vi "_Raise Nav Complete Event.vi"(4 "WebView2.lvlib:WebView2 Control.lvclass":refnum<class "WebView2 Control.lvclass">, 5 "Event Data":cluster{"sender":refnum<k24>, "e":refnum<k24>}, 6 "Control Ref":refnum<k24>, 7 "Event Common Data":T1) -> ()   [LabVIEW 2020, in "WebView2.lvlib" / "WebView2 Control.lvclass"]
uses:
  WebView2 Control.lvclass
  E:/Labview/LV 2023/PPL/PPL Builder/Libs/LV-WebView2/Source/Libs/Microsoft.Web.WebView2.Core.dll
  Libs/Microsoft.Web.WebView2.Core.dll
  WebView2 Control.lvclass/WebView2 Control.ctl
  WebView2 Event Filter Interface/WebView2 Event Filter Interface.lvclass
  Navigation Event Data.ctl
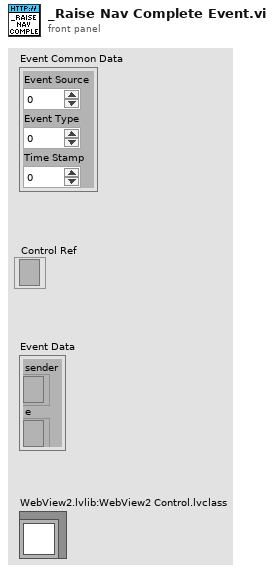
[diagram p1: front panel]
types:
  T1 = cluster{"Event Source":i32, "Event Type":u32, "Time Stamp":u32}
  T2 = typedef "WebView2.lvlib/WebView2 Control.lvclass/Navigation Event Data.ctl" = cluster{"HttpStatusCode":i32, "IsSuccess":bool, "NavigationId":u64, "WebErrorStatus":i32}
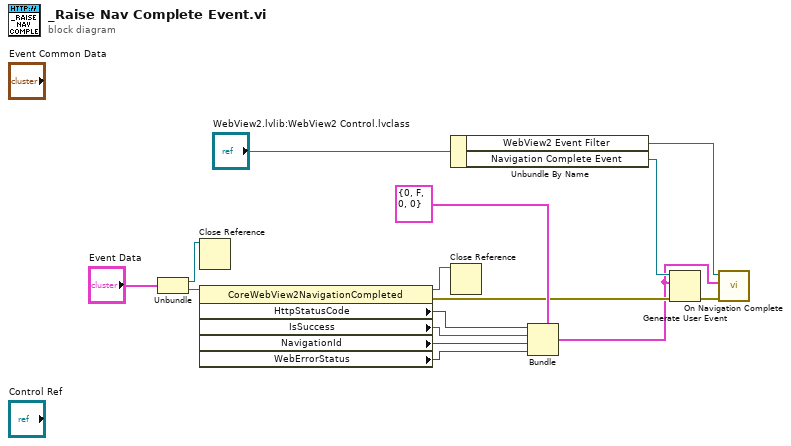
[diagram p0: block diagram]
diagram:
  n1 = Unbundle("Event Data") -> ("sender"=w5:refnum<k24>, "e"=w12:refnum<k24>)
  n2 = Close Reference(reference=w5) -> ()  [unwired: 1 in, 1 out]
  n3 = property class="CoreWebView2NavigationCompleted"(reference=w12) -> (reference out=w4:refnum<k24>, error out=w6:errorcluster, "HttpStatusCode"=w11:i32, "IsSuccess"=w10:bool, "NavigationId"=w9:u64, "WebErrorStatus"=w8:i32)  [unwired: 1 in]
  n4 = Unbundle By Name("WebView2.lvlib:WebView2 Control.lvclass") -> ("WebView2 Event Filter"=w1:refnum<class "WebView2 Event Filter Interface.lvclass">, "Navigation Complete Event"=w15:refnum<user-event>)
  n5 = Close Reference(reference=w4) -> ()  [unwired: 1 in, 1 out]
  n6 = Bundle(cluster=T2 {"HttpStatusCode"=0, "IsSuccess"=FALSE, "NavigationId"=0, "WebErrorStatus"=0} ("output cluster"), "HttpStatusCode"=w11, "IsSuccess"=w10, "NavigationId"=w9, "WebErrorStatus"=w8) -> (w2:T2)
  n7 = Generate User Event(user event=w15, event data cluster=w2, error in=w6) -> (error out=w3:errorcluster)  [unwired: 1 in, 1 out]
  n8 = call-dynamic "On Navigation Complete.vi"("error in (no error)"=w3, "Data"=w2, "WebView2 Event Filter Interface in"=w1) -> ()  [unwired: 8 in, 1 out]
